vi "Luminancia.vi"(5 "As (Area del OLED) cm2":dbl, 6 "S (Distancia OLED-fotodiodo) cm":dbl, 7 "Analog Vout":dbl, 8 "Respuesta fotopica (Cv)":dbl, 9 "Responsividad Normalizada (R)":dbl) -> (0 "Pin(W)":dbl, 2 "Luminancia (Cd/m2)":dbl, 3 "Iluminancia  lm/m2":dbl)   [LabVIEW 2020]
panel:
  # "m"
  # "2"
  # "m"
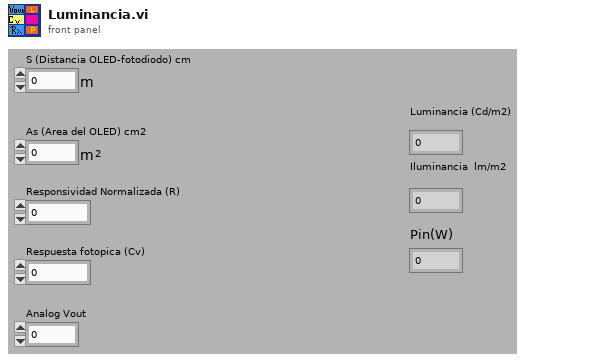
[diagram p1: front panel]
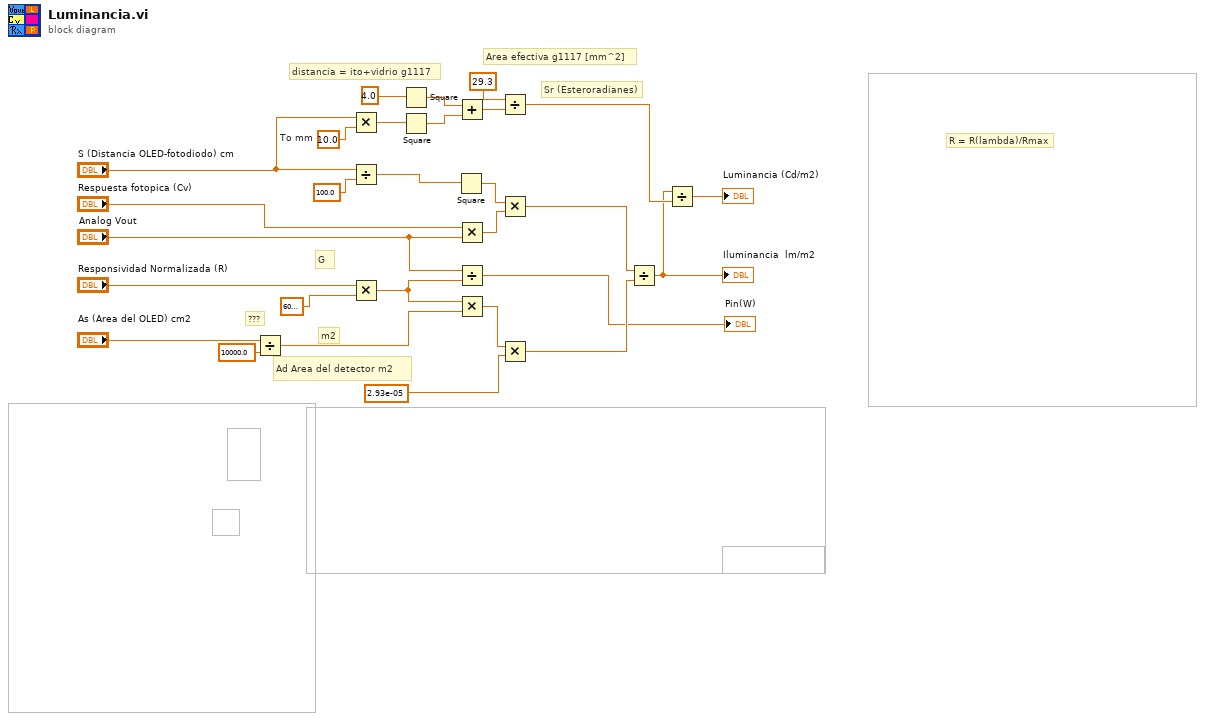
[diagram p0: block diagram]
diagram:
  w11 = 10.0  # To mm
  # "???"
  # "R = R(lambda)/Rmax"
  # "distancia = ito+vidrio g1117"
  # "Area efectiva g1117 [mm^2]"
  # "m2"
  # "Sr (Esteroradianes)"
  # "G"
  # "Ad Area del detector m2"
  n1 = Divide(x="As (Area del OLED) cm2", y=10000.0) -> (x/y=w4:dbl)
  n2 = Multiply(x="S (Distancia OLED-fotodiodo) cm", y=w11) -> (x*y=w12:dbl)
  n3 = Divide(x="S (Distancia OLED-fotodiodo) cm", y=100.0) -> (x/y=w9:dbl)
  n4 = Multiply(x="Responsividad Normalizada (R)", y=6000000.0) -> (x*y=w20:dbl)
  n5 = Square(x=4.0) -> (x^2=w17:dbl)
  n6 = Square(x=w12) -> (x^2=w16:dbl)
  n7 = Square(x=w9) -> (x^2=w27:dbl)
  n8 = Add(x=w17, y=w16) -> (x+y=w15:dbl)
  n9 = Multiply(x="Respuesta fotopica (Cv)", y="Analog Vout") -> (x*y=w28:dbl)
  n10 = Divide(x="Analog Vout", y=w20) -> (x/y=→"Pin(W)":dbl)
  n11 = Multiply(x=w20, y=w4) -> (x*y=w25:dbl)
  n12 = Divide(x=29.3 ("S"), y=w15) -> (x/y=w6:dbl)
  n13 = Multiply(x=w27, y=w28) -> (x*y=w26:dbl)
  n14 = Multiply(x=w25, y=2.93e-05) -> (x*y=w24:dbl)
  n15 = Divide(x=w26, y=w24) -> (x/y=w1:dbl)
  "Iluminancia  lm/m2" <- w1
  n16 = Divide(x=w1, y=w6) -> (x/y=→"Luminancia (Cd/m2)":dbl)
